vi "get lengths.vi"(8 "error in":errorcluster, 9 "Timeout (ms)":i32=-1, 11 "profibus reference":T2) -> (0 "error out":errorcluster, 2 "Slave Info List":T1(array[cluster]), 3 "profibus reference out":T2)   [LabVIEW 2013, in "dynamic profibus.lvlib"]
uses:
  dynamic profibus.lvlib
  fpga reference.ctl
  profibus master action.ctl
  <vilib>/rvi/interface/common/niFpgaWaitOnOcc.vi
  <vilib>/Utility/error.llb/Error Cluster From Error Code.vi
  <vilib>/rvi/errors/niLvFpgaAdjustHostInterfaceError.vi
  <vilib>/rvi/interface/nirviMethod/nirviMethod.xnode
  <vilib>/rvi/errors/niLvFpgaMergeErrorWithErrorCode.vi
  <vilib>/FPGAPlugInAG/Dynamic/niLvFpga_WriteFifo_Dynamic.vi
  <vilib>/FPGAPlugInAG/Dynamic/niLvFpga_ReadFifo_Dynamic.vi
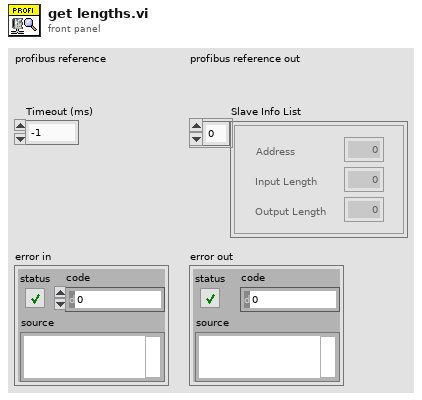
[diagram p1: front panel]
types:
  T1 = cluster{"Address":i8, "Input Length":u8, "Output Length":u8}[]
  T2 = typedef "dynamic profibus.lvlib/fpga reference.ctl" = refnum<k20>
  T3 = typedef "dynamic profibus.lvlib/profibus master action.ctl" = enum8{"initialize", "uninitialize", "stop", "get input", "get input size", "set output", "get output size", "get diagnostic", "transfer data", "transfer diagnostics", "read many inputs"}
  T4 = cluster{"Address":i8, "Input Length":u8, "Output Length":u8}
  T5 = typedef "dynamic profibus.lvlib/profibus master transmit header.ctl" = enum8{"Error", "Input", "Diagnostic", "input size", "output size", "many inputs"}
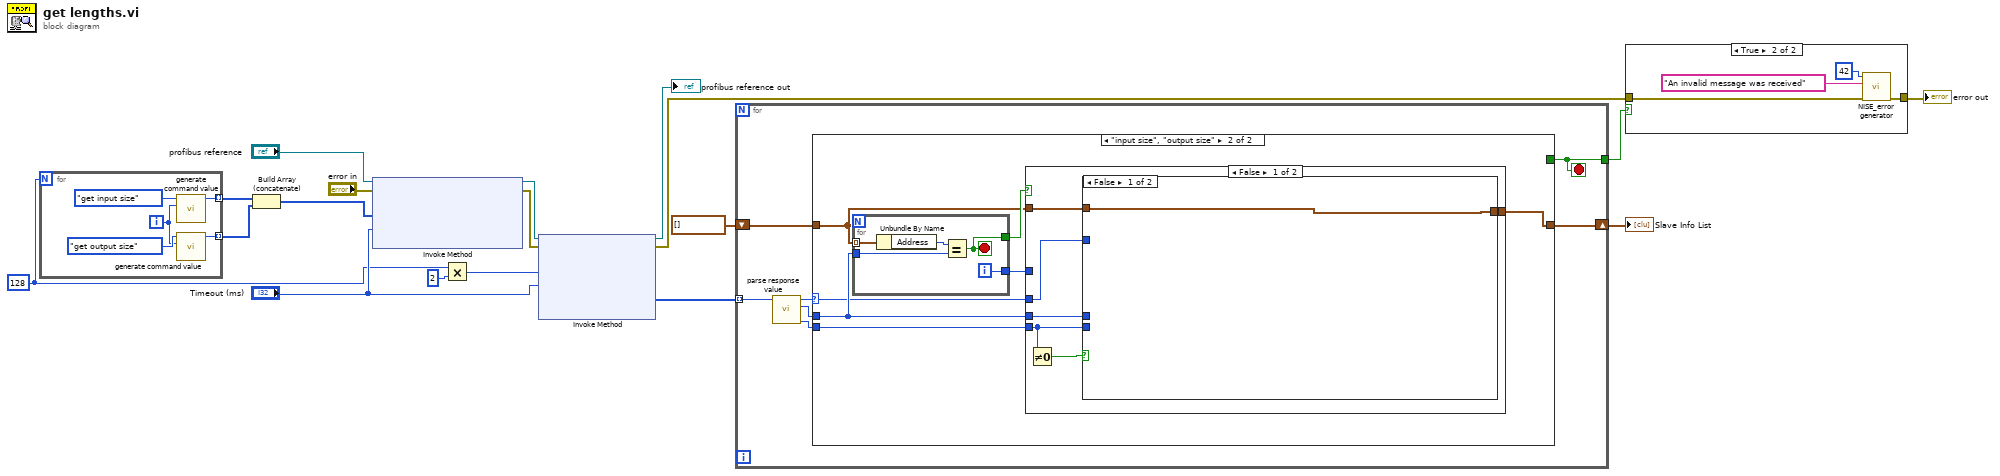
[diagram p0: block diagram]
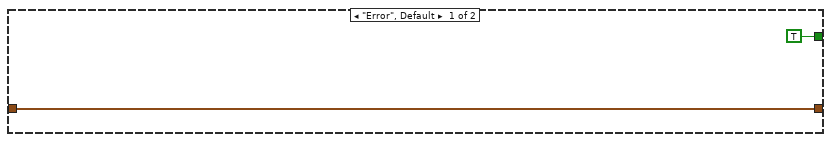
[diagram p3: hidden frame]
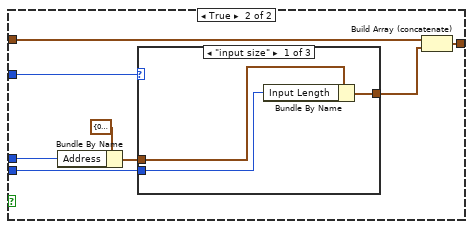
[diagram p4: hidden frame]
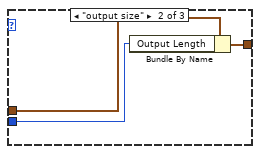
[diagram p5: hidden frame]
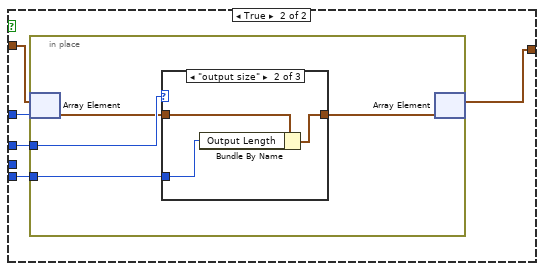
[diagram p7: hidden frame]
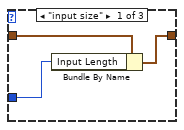
[diagram p8: hidden frame]
diagram:
  w2 = 128
  n1 = for {
    N: w2 -> [_]
    tunnel: [w21] -> w15 mode=indexing
    tunnel: [w20] -> w14 mode=indexing
    i -> [w19]
    n2 = call "generate command value.vi"("device"=w19, "action"=profibus_master_action."get input size") -> ("Element"=w20:u32)  [unwired: 9 in]
    n3 = call "generate command value.vi"("device"=w19, "action"=profibus_master_action."get output size") -> ("Element"=w21:u32)  [unwired: 9 in]
  }
  n4 = Build Array (concatenate)(w14, w15) -> (w11:u32[])
  n5 = xnode "Invoke Method"("FPGA VI Reference In"="profibus reference", "error in"="error in", "Data"=w11, "Timeout (ms)"="Timeout (ms)") -> ("FPGA VI Reference Out"=w13:T2, "error out"=w17:errorcluster)  [unwired: 1 out]
  n6 = Multiply(x=w2, y=2) -> (x*y=w3:i32)
  n7 = xnode "Invoke Method"("FPGA VI Reference In"=w13, "error in"=w17, "Number of Elements"=w3, "Timeout (ms)"="Timeout (ms)") -> ("FPGA VI Reference Out"=→"profibus reference out":T2, "error out"=w5:errorcluster, "Data"=w9:u32[])  [unwired: 1 out]
  n8 = for {
    tunnel: w9 -> [w30] mode=indexing
    shift-right: [w25] -> w7
    shift-left: T1 [] ("Slave Info List") -> [w26]
    tunnel: [w24] -> w6
    stop <- w24 stop-if-true
    n9 = call "parse response value.vi"("Element"=w30) -> ("data"=w27:u8, "device"=w28:u8, "header"=w29:T5)  [unwired: 7 in, 1 out]
    n10 = case shown="\"input size\", \"output size\"" w29 {
      selector: w29 -> [_ w33]
      tunnel: w28 -> [_ w35]
      tunnel: w27 -> [_ w34]
      tunnel: w26 -> [w32 w37]
      tunnel: [w32 w36] -> w25
      tunnel: [TRUE _] -> w24
      frame "Error", Default {
      }
      frame "input size", "output size" {
        n11 = for {
          tunnel: w37 -> [w82] mode=indexing
          tunnel: w35 -> [w80]
          tunnel: [w78] -> w39
          tunnel: [w79] -> w38
          i -> [w79]
          stop <- w78 stop-if-true
          n12 = Unbundle By Name(w82) -> ("Address"=w81:i8)
          n13 = Equal?(x=w81, y=w80) -> (x = y?=w78:bool)
        }
        n14 = case shown="False" w39 {
          tunnel: w38 -> [_ w66]
          tunnel: w37 -> [w45 w65]
          tunnel: [w44 w64] -> w36
          tunnel: w35 -> [w43 _]
          tunnel: w34 -> [w41 w62]
          tunnel: w33 -> [w42 w63]
          frame False {
            n15 = Not Equal To 0?(x=w41) -> (x != 0?=w40:bool)
            n16 = case shown="False" w40 {
              tunnel: w45 -> [w46 w54]
              tunnel: [w46 w53] -> w44
              tunnel: w43 -> [_ w51]
              tunnel: w42 -> [_ w50]
              tunnel: w41 -> [_ w47]
              frame False {
              }
              frame True {
                n17 = Bundle By Name(cluster=T4 {"Address"=0, "Input Length"=0, "Output Length"=0} ("Slave Info"), "Address"=w51) -> (w49:T4)
                n18 = case shown="\"input size\"" w50 {
                  tunnel: w49 -> [w57 w60 w61]
                  tunnel: [w56 w59 w61] -> w48
                  tunnel: w47 -> [w55 w58 _]
                  frame "input size" {
                    n19 = Bundle By Name(cluster=w57, "Input Length"=w55) -> (w56:T4)
                  }
                  frame "output size" {
                    n20 = Bundle By Name(cluster=w60, "Output Length"=w58) -> (w59:T4)
                  }
                  frame Default {
                  }
                }
                n21 = Build Array (concatenate)(w54, w48) -> (w53:T1)
              }
            }
          }
          frame True {
            n22 = in-place {
              in-place-border: w63 -> [w70]
              in-place-border: w62 -> [w67]
              n23 = in-place-array #1(w65, w66) -> (w69:T4)
              n24 = case shown="\"output size\"" w70 {
                tunnel: w69 -> [w73 w76 w77]
                tunnel: [w72 w75 w77] -> w68
                tunnel: w67 -> [w71 w74 _]
                frame "input size" {
                  n25 = Bundle By Name(cluster=w73, "Input Length"=w71) -> (w72:T4)
                }
                frame "output size" {
                  n26 = Bundle By Name(cluster=w76, "Output Length"=w74) -> (w75:T4)
                }
                frame Default {
                }
              }
              n27 = in-place-array #1(w68) -> (w64:T1)  [unwired: 1 out]
            }
          }
        }
      }
    }
  }
  "Slave Info List" <- w7
  n28 = case shown="True" w6 {
    tunnel: w5 -> [w83 w87]
    tunnel: [w83 w86] -> w4
    frame False {
    }
    frame True {
      n29 = call <vilib>:"NISE_error generator.vi"("error in"=w87, "append error message"="An invalid message was received", "error code (0)"=42) -> ("error out"=w86:errorcluster)  [unwired: 6 in]
    }
  }
  "error out" <- w4
